vi "virtual sheet (shared buffer).vi"() -> ()   [LabVIEW 2020]
uses:
  HW Timed SPIM/HW Timed SPIM/DAQ Timed SPIM.lvclass
  C:/Program Files/National Instruments/LabVIEW 2020/vi.lib/ActorFramework/Actor/Actor.lvclass
  HW Timed SPIM/HamamatsuFluor_v2/HamamatsuFluor/HamamatsuFluor.lvclass
  C:/WormSPIM/Labview2/SPIM Engine/HW Timed SPIM/Abstract DAQ Triggered Actor/Abstract DAQ Triggered Actor.lvclass
  HW Timed SPIM/DAQ Timed SPIM Messages/Add Camera Msg/Add Camera Msg.lvclass/Add Camera Msg.ctl
  <vilib>/ActorFramework/Message Enqueuer/Message Enqueuer.lvclass/Message Enqueuer.ctl
  <vilib>/ActorFramework/Reply Msg/Reply Msg.lvclass/Reply Msg.ctl
  HW Timed SPIM/HamamatsuFluor_v2/HamamatsuFluor Messages/Set ROI v2 Msg/Set ROI v2 Msg.lvclass/Set ROI v2 Msg.ctl
  HW Timed SPIM/HamamatsuFluor_v2/HamamatsuFluor Messages/Set Buffer Length Msg/Set Buffer Length Msg.lvclass/Set Buffer Length Msg.ctl
  HW Timed SPIM/HamamatsuFluor_v2/HamamatsuFluor Messages/Set Exposure Msg/Set Exposure Msg.lvclass/Set Exposure Msg.ctl
  HW Timed SPIM/Abstract DAQ Triggered Actor Messages/Set Save Directory Msg/Set Save Directory Msg.lvclass/Set Save Directory Msg.ctl
  HW Timed SPIM/DAQ Timed SPIM Messages/Set Main Loop Data Msg/Set Main Loop Data Msg.lvclass/Set Main Loop Data Msg.ctl
  HW Timed SPIM/DAQ Timed SPIM Messages/Set Warmup Data Msg/Set Warmup Data Msg.lvclass/Set Warmup Data Msg.ctl
  HW Timed SPIM/DAQ Timed SPIM Messages/Set Cooldown Data Msg/Set Cooldown Data Msg.lvclass/Set Cooldown Data Msg.ctl
  <vilib>/ActorFramework/Message Enqueuer/Enqueue.vi
  <vilib>/ActorFramework/Reply Msg/Send Message And Wait For Response.vi
  HW Timed SPIM/DAQ Timed SPIM Messages/Add Camera Msg/Add Camera Msg.lvclass
  C:/Program Files/National Instruments/LabVIEW 2020/vi.lib/ActorFramework/Message/Message.lvclass
  HW Timed SPIM/DAQ Timed SPIM Messages/Get Device Enqueuers Msg/Get Device Enqueuers Msg.lvclass
  C:/Program Files/National Instruments/LabVIEW 2020/vi.lib/ActorFramework/Reply Msg/Reply Msg.lvclass
  <vilib>/ActorFramework/Reply Msg/Reply Msg.lvclass
  HW Timed SPIM/HamamatsuFluor_v2/HamamatsuFluor Messages/Set ROI v2 Msg/Set ROI v2 Msg.lvclass
  HW Timed SPIM/HamamatsuFluor_v2/HamamatsuFluor Messages/Set Buffer Length Msg/Set Buffer Length Msg.lvclass
  HW Timed SPIM/HamamatsuFluor_v2/HamamatsuFluor Messages/Set Exposure Msg/Set Exposure Msg.lvclass
  HW Timed SPIM/Abstract DAQ Triggered Actor Messages/Set Save Directory Msg/Set Save Directory Msg.lvclass
  HW Timed SPIM/DAQ Timed SPIM Messages/Launch Basic Controller Msg/Launch Basic Controller Msg.lvclass
  <vilib>/ActorFramework/Stop Msg/Stop Msg.lvclass
  HW Timed SPIM/DAQ Timed SPIM Messages/Set Main Loop Data Msg/Set Main Loop Data Msg.lvclass
  HW Timed SPIM/DAQ Timed SPIM Messages/Set Warmup Data Msg/Set Warmup Data Msg.lvclass
  HW Timed SPIM/DAQ Timed SPIM Messages/Set Cooldown Data Msg/Set Cooldown Data Msg.lvclass
  <vilib>/ActorFramework/Message Priority Queue/Priority Enqueue.vi
  <vilib>/ActorFramework/Message Enqueuer/Message Enqueuer.lvclass
  <vilib>/ActorFramework/Actor/Actor.lvclass
  <resource>/objmgr/daqmx.rc
  Scan generators/Scan Generators.lvlib
panel:
  in  "overshoot time (ms) (applied twice)":dbl=0.3
  out "Readout time":dbl
  in  "Line Exposure (ms)":dbl=0.05
  out "error out":errorcluster
  in  "error in (no error)":errorcluster
  in  "Z Slices":cluster{"start":dbl, "delta":dbl, "end":dbl}={"start"=100.0, "delta"=-1.355, "end"=20.0}
  in  "Signal delays":T1={"ETL delay (samples)"=10, "Scanner delay (samples)"=-102, "Laser delay (samples)"=7}
  in  "Volume period (s)":dbl=0.3
  in  "Frame period (s)":dbl=0.004
  in  "Laser exposure (s)":dbl=0.00025
  in  "Scanner calibration":cluster{"Offset":dbl, "Amplitude":dbl}[](array[cluster])=[{"Offset"=2.5299999999999994, "Amplitude"=-0.32}, {"Offset"=2.225, "Amplitude"=0.43}, {"Offset"=2.5, "Amplitude"=0.0}, {"Offset"=2.37, "Amplitude"=0.0}] {"Amplitude" min=-5.0 max=5.0 step=0.005; "Offset" min=0.0 max=5.0 step=0.005}
  in  "ROI":T2={"Horizontal Offset"=256, "Vertical Offset"=896, "Horizontal Size"=1536, "Vertical Size"=256}
  in  "Path":path=path "E:/"
  in  "stop":bool
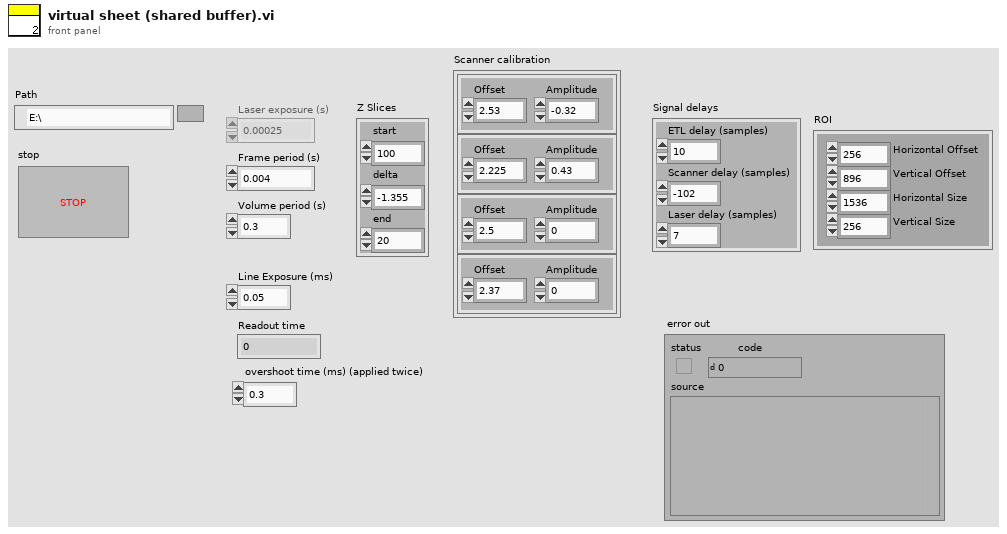
[diagram p1: front panel]
types:
  T1 = cluster{"ETL delay (samples)":i32, "Scanner delay (samples)":i32, "Laser delay (samples)":i32}
  T2 = cluster{"Horizontal Offset":i32, "Vertical Offset":i32, "Horizontal Size":i32, "Vertical Size":i32}
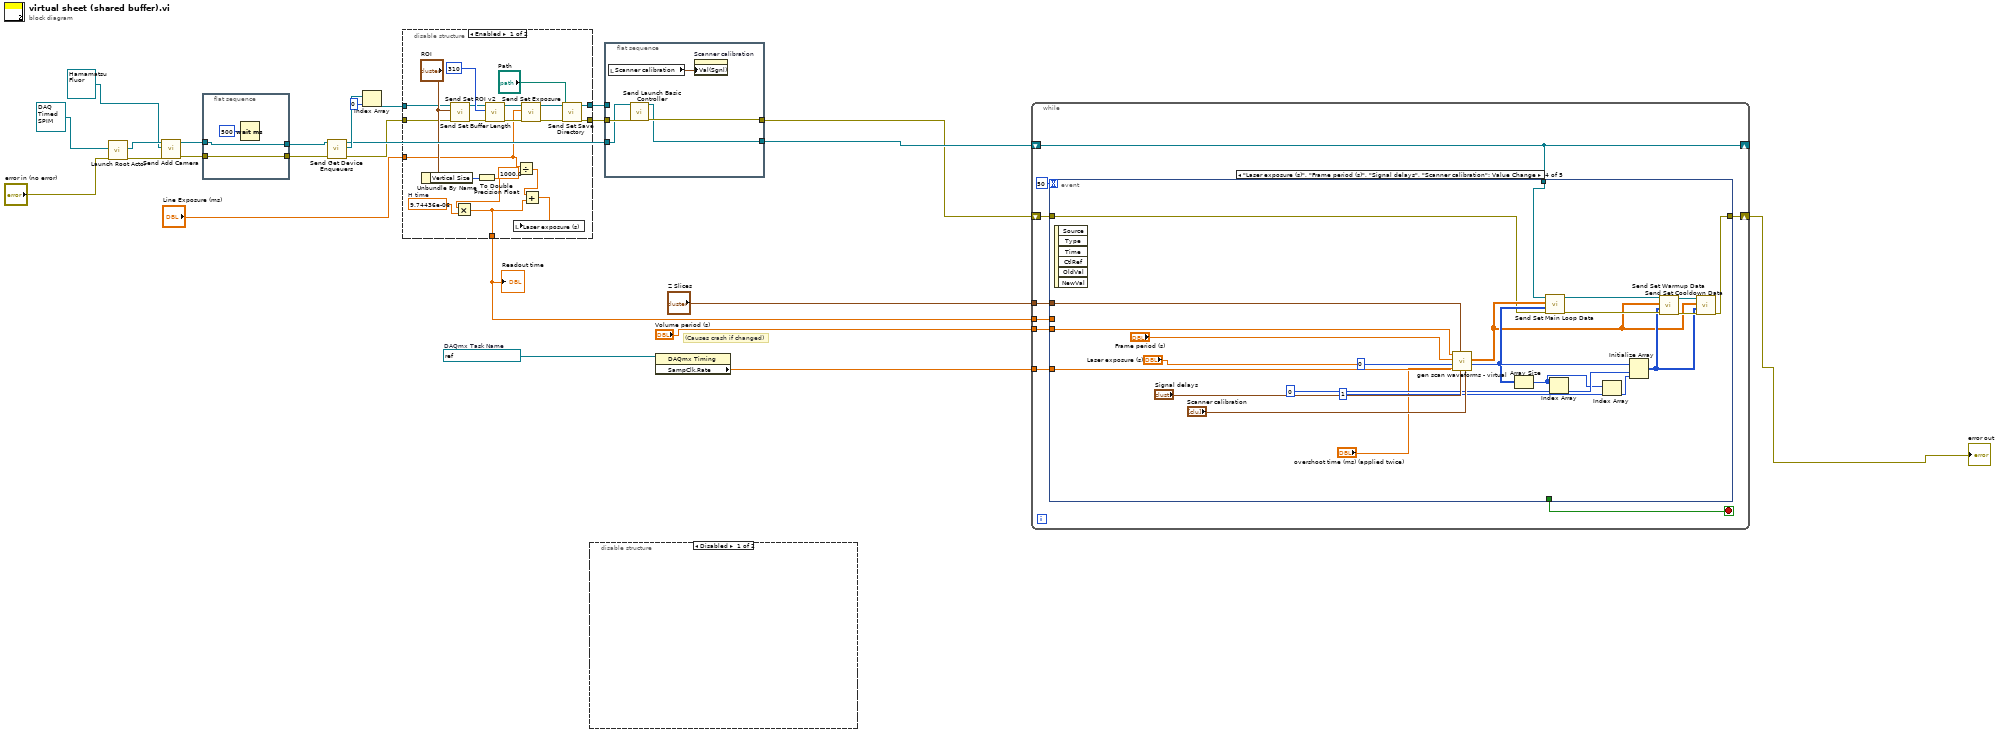
[diagram p0: block diagram]
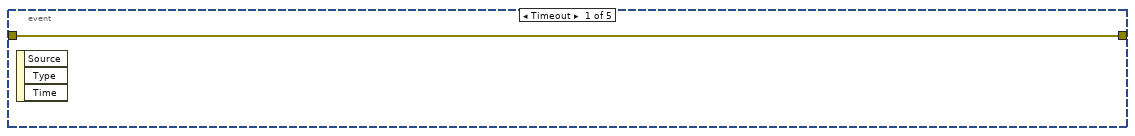
[diagram p4: hidden frame]
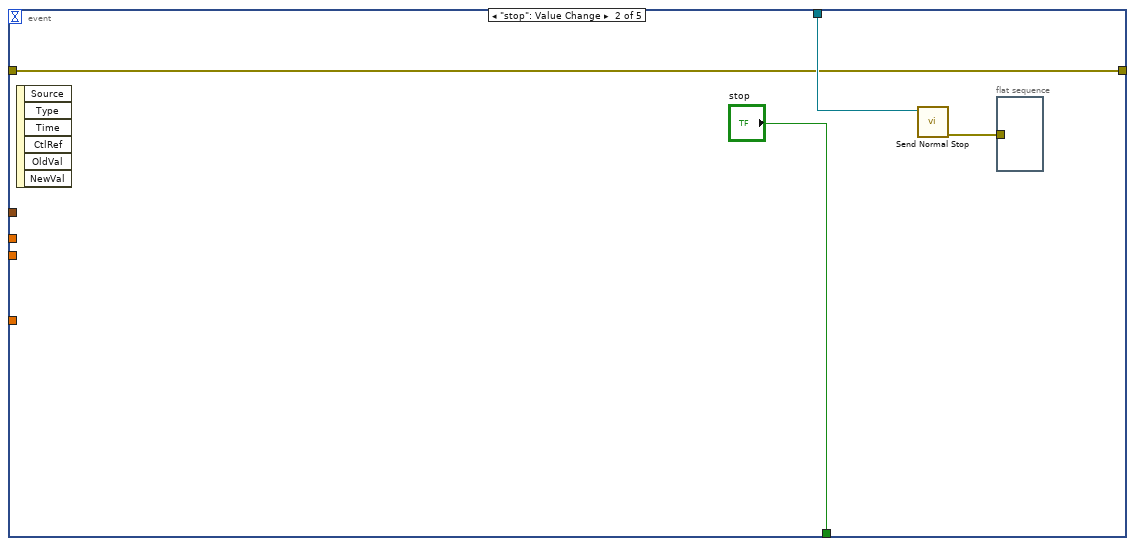
[diagram p5: hidden frame]
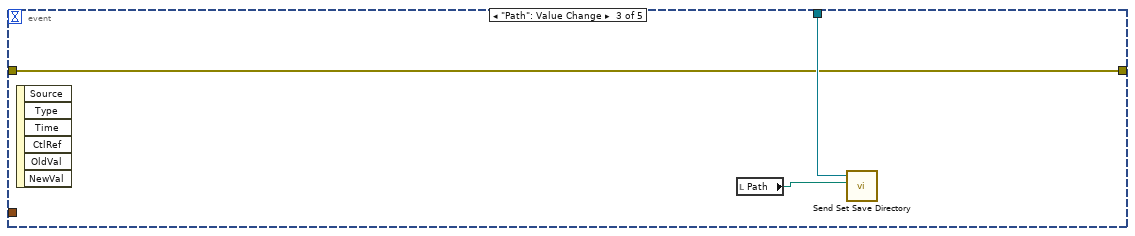
[diagram p6: hidden frame]
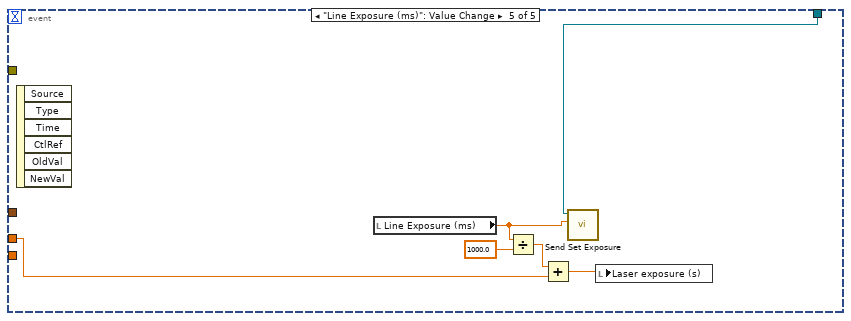
[diagram p7: hidden frame]
diagram:
  w22 = refnum<k21> "SPIM_Analog_Task"  # DAQmx Task Name
  # "(Causes crash if changed)"
  n1 = call <vilib>:"Launch Root Actor.vi"("error in (no error)"="error in (no error)", "Actor"=refnum<class "DAQ Timed SPIM.lvclass"> refnum ("DAQ Timed SPIM.lvlib:DAQ Timed SPIM.lvclass")) -> ("error out"=w23:errorcluster, "Actor's Enqueuer"=w24:refnum<class "Message Enqueuer.lvclass">)  [unwired: 8 in]
  n2 = call "Send Add Camera.vi"("error in (no error)"=w23, "DAQ Timed Camera"=refnum<class "HamamatsuFluor.lvclass"> refnum ("DAQ Timed SPIM.lvlib:HamamatsuFluor_v2.lvlib:HamamatsuFluor.lvclass"), "Message Enqueuer"=w24) -> ("error out"=w2:errorcluster, "Message Enqueuer out"=w4:refnum<class "Message Enqueuer.lvclass">)  [unwired: 7 in]
  n3 = flat-sequence {
    tunnel: w4 -> [w27]
    tunnel: [w27] -> w3
    tunnel: w2 -> [w26]
    tunnel: [w26] -> w1
    frame #0 {
      n4 = Wait (ms)(milliseconds to wait=u32 500) -> ()  [unwired: 1 out]
    }
  }
  n5 = call "Send Get Device Enqueuers.vi"("error in (no error)"=w1, "Message Enqueuer"=w3) -> ("error out"=w9:errorcluster, "Camera Enqueuers"=w21:refnum<class "Message Enqueuer.lvclass">[], "Message Enqueuer out"=w16:refnum<class "Message Enqueuer.lvclass">)  [unwired: 6 in, 1 out]
  n6 = Index Array(array=w21, index=0) -> (element=w10:refnum<class "Message Enqueuer.lvclass">)
  n7 = disable-structure shown="Enabled" {
    disable-tunnel: [w49 w50] -> w12
    disable-tunnel: [w48 w51] -> w11
    disable-tunnel: w10 -> [w30 w51]
    disable-tunnel: w9 -> [w29 w50]
    disable-tunnel: "Line Exposure (ms)" -> [w32 _]
    disable-tunnel: [w34 _] -> w5
    frame Enabled {
      w40 = 9.74436e-06  # H time
      n8 = Unbundle By Name("ROI") -> ("Vertical Size"=w42:i32)
      n9 = call "Send Set ROI v2.vi"("error in (no error)"=w29, "ROI"="ROI", "Message Enqueuer"=w30) -> ("error out"=w44:errorcluster, "Message Enqueuer out"=w45:refnum<class "Message Enqueuer.lvclass">)  [unwired: 7 in]
      n10 = To Double Precision Float(number=w42) -> (double precision float=w41:dbl)
      n11 = Multiply(x=w41, y=w40) -> (x*y=w34:dbl)
      n12 = call "Send Set Buffer Length.vi"("error in (no error)"=w44, "Buffer Size"=310, "Message Enqueuer"=w45) -> ("error out"=w39:errorcluster, "Message Enqueuer out"=w38:refnum<class "Message Enqueuer.lvclass">)  [unwired: 7 in]
      n13 = Divide(x=w32, y=1000.0) -> (x/y=w33:dbl)
      n14 = call "Send Set Exposure.vi"("error in (no error)"=w39, "Line exposure (ms)"=w32, "Message Enqueuer"=w38) -> ("error out"=w37:errorcluster, "Message Enqueuer out"=w36:refnum<class "Message Enqueuer.lvclass">)  [unwired: 7 in]
      n15 = Add(x=w33, y=w34) -> (x+y=w35:dbl)
      n16 = local write "Laser exposure (s)"(w35) -> ()
      n17 = call "Send Set Save Directory.vi"("error in (no error)"=w37, "Path"="Path", "Message Enqueuer"=w36) -> ("error out"=w49:errorcluster, "Message Enqueuer out"=w48:refnum<class "Message Enqueuer.lvclass">)  [unwired: 7 in]
    }
    frame Disabled {
    }
  }
  "Readout time" <- w5
  n18 = disable-structure shown="Disabled" {
    frame Disabled {
    }
    frame Enabled {
    }
  }
  n19 = flat-sequence {
    tunnel: w12 -> [w55]
    tunnel: [w54] -> w8
    tunnel: w11 -> [_]
    tunnel: w16 -> [w53]
    tunnel: [w52] -> w15
    frame #0 {
      n20 = local read "Scanner calibration"() -> (w56:cluster{"Offset":dbl, "Amplitude":dbl}[])
      n21 = call "Send Launch Basic Controller.vi"("error in (no error)"=w55, "Message Enqueuer"=w53) -> ("error out"=w54:errorcluster, "Message Enqueuer out"=w52:refnum<class "Message Enqueuer.lvclass">)  [unwired: 8 in]
      n22 = property on="Scanner calibration" class="Arr (strict)"("Val(Sgnl)"=w56) -> ()  [unwired: 2 in, 2 out]
    }
  }
  n23 = property class="DAQmx Timing"(reference=w22) -> ("SampClk.Rate"=w19:dbl)  [unwired: 1 in, 2 out]
  n24 = while {
    shift-right: [w64] -> _
    shift-left: w15 -> [w64]
    tunnel: w19 -> [w63]
    tunnel: "Z Slices" -> [w62]
    tunnel: "Volume period (s)" -> [w61]
    shift-right: [w58] -> w7
    shift-left: w8 -> [w59]
    tunnel: w5 -> [w57]
    stop <- w65 stop-if-true
    n25 = event shown="[3] \"Laser exposure (s)\", \"Frame period (s)\", \"Signal delays\", \"Scanner calibration\": Value Change" {
      selector: _ -> [_ _ _ _ _]
      dyn-events: _ -> [_ _ _ _ _]
      timeout: 50 -> [_ _ _ _ _]
      tunnel: [_ "stop" _ _ _] -> w65
      tunnel: w64 -> [_ w69 w73 w84 w103]
      tunnel: w63 -> [_ _ _ w87 _]
      tunnel: w62 -> [_ _ _ w78 _]
      tunnel: w61 -> [_ _ _ w77 _]
      tunnel: w59 -> [w66 w67 w71 w76 _]
      tunnel: [w66 w67 w71 w75 _] -> w58
      tunnel: w57 -> [_ _ _ _ w99]
      event Timeout {
        n26 = event-data() -> ()  [unwired: 1 in, 3 out]
      }
      event "stop": Value Change {
        n27 = event-data() -> ()  [unwired: 1 in, 6 out]
        n28 = call <vilib>:"Send Normal Stop.vi"("Message Enqueuer"=w69) -> ("error out"=w68:errorcluster)  [unwired: 10 in]
        n29 = flat-sequence {
          tunnel: w68 -> [_]
          frame #0 {
          }
        }
      }
      event "Path": Value Change {
        n30 = event-data() -> ()  [unwired: 1 in, 6 out]
        n31 = local read "Path"() -> (w72:path)
        n32 = call "Send Set Save Directory.vi"("Path"=w72, "Message Enqueuer"=w73) -> ()  [unwired: 8 in, 2 out]
      }
      event "Laser exposure (s)", "Frame period (s)", "Signal delays", "Scanner calibration": Value Change {
        n33 = event-data() -> ()  [unwired: 1 in, 6 out]
        n34 = call "gen scan waveforms - virtual.vi"("overshoot time (ms) (applied twice)"="overshoot time (ms) (applied twice)", "Scanner calibration"="Scanner calibration", "Signal delays"="Signal delays", "Z Slices"=w78, "AO sample rate"=w87, "Flash duration (s)"="Laser exposure (s)", "frame period (s)"="Frame period (s)", "volume period (s)"=w77) -> ("Digital signals"=w83:u8[][], "Analog signals"=w79:dbl[][])  [unwired: 2 in]
        n35 = Array Size(array=w83) -> (size(s)=w90:i32[])
        n36 = call "Send Set Main Loop Data.vi"("error in (no error)"=w76, "Digital"=w83, "Analog"=w79, "Message Enqueuer"=w84) -> ("error out"=w81:errorcluster, "Message Enqueuer out"=w82:refnum<class "Message Enqueuer.lvclass">)  [unwired: 6 in]
        n37 = Index Array(array=w90, index=0) -> (element=w91:i32)
        n38 = Index Array(array=w90, index=1) -> (element=w88:i32)
        n39 = Initialize Array(u8 0, w91, w88) -> (w80:u8[][])
        n40 = call "Send Set Warmup Data.vi"("error in (no error)"=w81, "Digital"=w80, "Analog"=w79, "Message Enqueuer"=w82) -> ("error out"=w85:errorcluster, "Message Enqueuer out"=w86:refnum<class "Message Enqueuer.lvclass">)  [unwired: 6 in]
        n41 = call "Send Set Cooldown Data.vi"("error in (no error)"=w85, "Digital"=w80, "Analog"=w79, "Message Enqueuer"=w86) -> ("error out"=w75:errorcluster)  [unwired: 6 in, 1 out]
      }
      event "Line Exposure (ms)": Value Change {
        n42 = event-data() -> ()  [unwired: 1 in, 6 out]
        n43 = local read "Line Exposure (ms)"() -> (w102:dbl)
        n44 = Divide(x=w102, y=1000.0) -> (x/y=w100:dbl)
        n45 = Add(x=w100, y=w99) -> (x+y=w98:dbl)
        n46 = call "Send Set Exposure.vi"("Line exposure (ms)"=w102, "Message Enqueuer"=w103) -> ()  [unwired: 8 in, 2 out]
        n47 = local write "Laser exposure (s)"(w98) -> ()
      }
    }
  }
  "error out" <- w7
